vi "lib path.vi"() -> (3 "lib path":path)   [LabVIEW 2023, in "xnet_canopen.lvlib"]
uses:
  xnet_canopen.lvlib
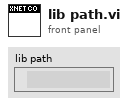
[diagram p1: front panel]
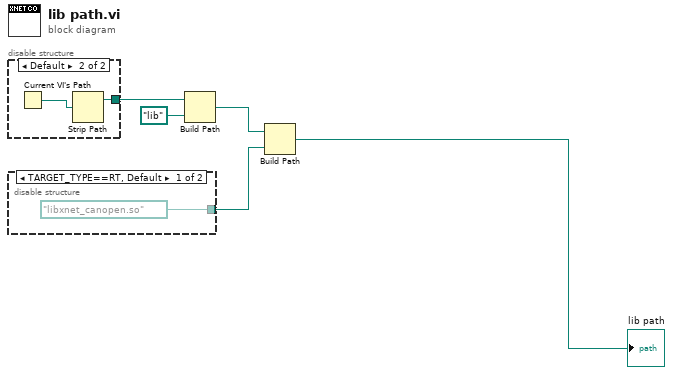
[diagram p0: block diagram]
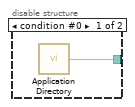
[diagram p2: hidden frame]
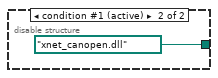
[diagram p3: hidden frame]
diagram:
  n1 = disable-structure shown="Default" {
    disable-tunnel: [w6 w7] -> w1
    frame condition #0 {
      n2 = call <vilib>:"Application Directory.vi"() -> ("Application Directory"=w6:path)
    }
    frame condition #1 (active) {
      n3 = Current VI's Path() -> (path=w8:path)
      n4 = Strip Path(path=w8) -> (stripped path=w7:path)  [unwired: 1 out]
    }
  }
  n5 = disable-structure shown="TARGET_TYPE==RT, Default" {
    disable-tunnel: [path "libxnet_canopen.so" ("path in") path "xnet_canopen.dll" ("path in")] -> w4
    frame condition #0 {
    }
    frame condition #1 (active) {
    }
  }
  n6 = Build Path(base path=w1, name or relative path=path "lib") -> (appended path=w3:path)
  n7 = Build Path(base path=w3, name or relative path=w4) -> (appended path=→"lib path":path)
